vi "get asset.vi"(10 "Asset RID":string, 11 "connection":refnum<class "Nominal Client.lvclass">) -> (0 "error out":errorcluster, 3 "Asset":refnum<class "asset.lvclass">)   [LabVIEW 2020, in "nominal core steps.lvlib"]
doc: "Look up an asset object by RID.\n<b> </b> <b> </b>"
uses:
  nominal core steps.lvlib
  <vilib>/Nominal/Nominal IO Client/lv_src/Nominal Client/Nominal Client.lvclass
  <vilib>/Nominal/Nominal IO Client/lv_src/asset/asset.lvclass
  <vilib>/Nominal/Nominal IO Client/lv_src/Nominal Client/asset.get.vi
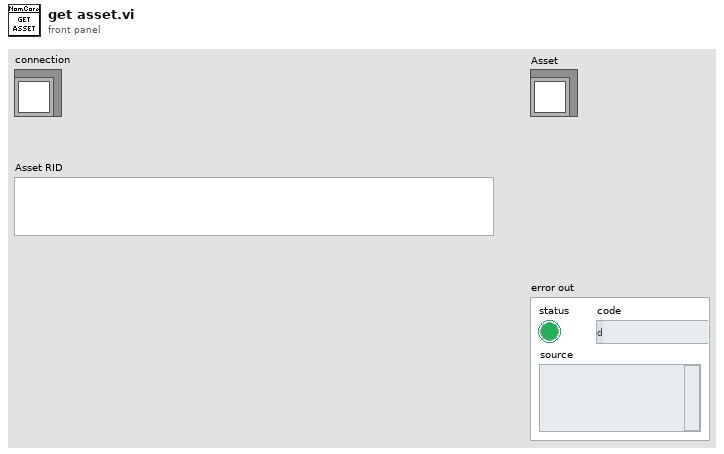
[diagram p1: front panel]
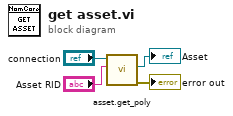
[diagram p0: block diagram]
diagram:
  n1 = call-poly <vilib>:"asset.get_poly.vi"("Asset RID"="Asset RID", "Nominal Client in"="connection") -> ("error out"=→"error out":errorcluster, "Asset"=→"Asset":refnum<class "asset.lvclass">)  [unwired: 7 in, 1 out]
